vi "Insert_database.vi"(6 "data":variant, 7 "create table? (F)":bool, 8 "error in (no error)":errorcluster caption="错误输入（无错误）", 9 "columns":string[](array[string]), 10 "table":string, 11 "Database_access 输入":refnum<class "Database_access.lvclass">) -> (0 "error out":errorcluster caption="错误输出", 3 "Database_access 输出":refnum<class "Database_access.lvclass">)   [LabVIEW 2025, in "Database_access.lvclass"]
uses:
  Database_access.lvclass
  Database_access.lvclass/Database_access.ctl
  <vilib>/addons/database/NI_Database_API.lvlib
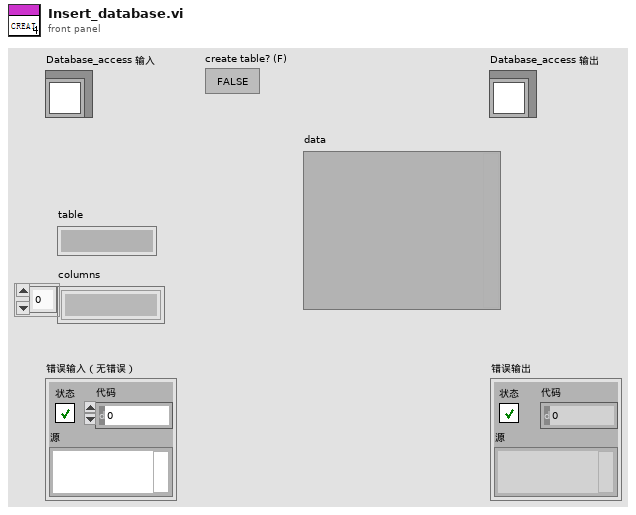
[diagram p1: front panel]
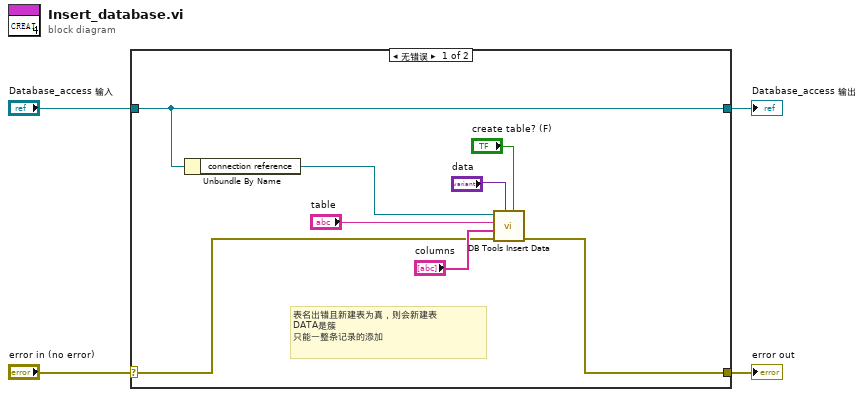
[diagram p0: block diagram]
diagram:
  n1 = case shown="无错误" "error in (no error)" {
    selector: "error in (no error)" -> [w7 w14]
    tunnel: [w6 w14] -> w3
    tunnel: [w12 w13] -> w1
    tunnel: "Database_access 输入" -> [w12 w13]
    frame No Error {
      # "表名出错且新建表为真，则会新建表\nDATA是簇\n只能一整条记录的添加"
      n2 = Unbundle By Name(w12) -> ("connection reference"=w11:refnum<k1>)
      n3 = call <vilib>:"DB Tools Insert Data.vi"("create table? (F)"="create table? (F)", "data"="data", "error in (no error)"=w7, "columns"="columns", "table"="table", "connection reference"=w11) -> ("error out"=w6:errorcluster)  [unwired: 4 in, 1 out]
    }
    frame Error {
    }
  }
  "error out" <- w3
  "Database_access 输出" <- w1
